vi "Replace Default with Tag.vi"(5 "instance id":string, 7 "engine configuration in":refnum<class "engine configuration.lvclass">, 9 "Channel Index":i32, 10 "Channel":refnum<class "TBM channel.lvclass">, 11 "Array in":string[](array[string])) -> (3 "Array out":string[](array[string]))   [LabVIEW 2015, in "PID Module configuration.lvclass"]
uses:
  module/configuration/PID Module configuration.lvclass
  <vilib>/NI/Module Execution Interface/Engine Configuration/engine configuration.lvclass
  <vilib>/NI/Tag Bus Module Framework/channel/TBM channel.lvclass
  <vilib>/NI/Module Execution Interface/Engine Configuration/unique channel identifier.ctl
  <vilib>/NI/Tag Bus/tag/tag descriptor.lvclass/tag descriptor.ctl
  <vilib>/NI/Module Execution Interface/Engine Configuration/engine configuration.lvclass/engine configuration.ctl
  <vilib>/NI/Tag Bus/tag/tag descriptor.lvclass
panel:
  out "readers":T1[](array[typedef])
  out "writer":T1
  out "Array":string[](array[string])
  out "name":string
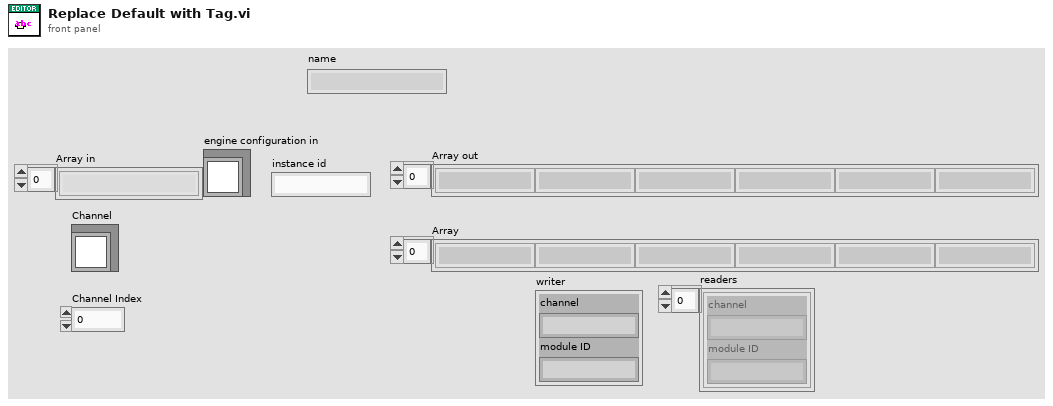
[diagram p1: front panel]
types:
  T1 = typedef "engine configuration.lvclass/unique channel identifier.ctl" = cluster{"channel":string, "module ID":string}
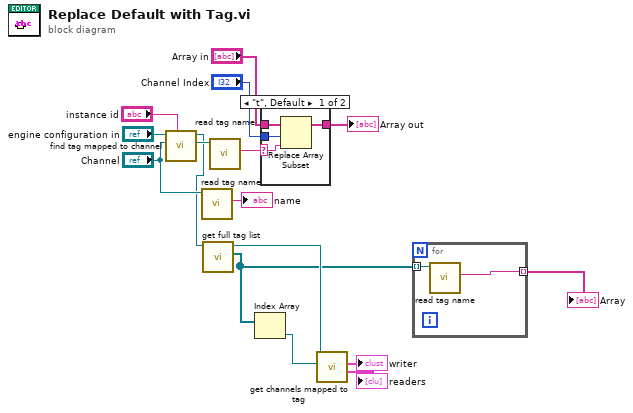
[diagram p0: block diagram]
diagram:
  n1 = call <vilib>:"find tag mapped to channel.vi"("owner"="instance id", "channel"="Channel", "engine configuration in"="engine configuration in") -> ("tag"=w15:refnum<class "tag descriptor.lvclass">, "engine configuration out"=w7:refnum<class "engine configuration.lvclass">)  [unwired: 6 in, 1 out]
  n2 = call <vilib>:"read tag name.vi"("system tag in"="Channel") -> ("name"=→"name":string)  [unwired: 8 in, 2 out]
  n3 = call <vilib>:"get full tag list.vi"("engine configuration in"=w7) -> ("tag list"=w4:refnum<class "tag descriptor.lvclass">[], "engine configuration out"=w5:refnum<class "engine configuration.lvclass">)  [unwired: 9 in]
  n4 = call <vilib>:"read tag name.vi"("system tag in"=w15) -> ("name"=w13:string)  [unwired: 8 in, 2 out]
  n5 = Index Array(array=w4) -> (element=w3:refnum<class "tag descriptor.lvclass">)  [unwired: 1 in]
  n6 = case shown="\"t\", Default" w13 {
    selector: w13 -> [w20 _]
    tunnel: [w18 w21] -> w12
    tunnel: "Array in" -> [w19 w21]
    tunnel: "Channel Index" -> [w17 _]
    frame "t", Default {
      n7 = Replace Array Subset(array=w19, new element=w20, index=w17) -> (w18:string[])
    }
    frame "" {
    }
  }
  "Array out" <- w12
  n8 = call-dynamic "get channels mapped to tag.vi"("tag"=w3, "engine configuration in"=w5) -> ("readers"=→"readers":T1[], "writer"=→"writer":T1)  [unwired: 6 in, 2 out]
  n9 = for {
    tunnel: w4 -> [w23] mode=indexing
    tunnel: [w22] -> w6 mode=indexing
    n10 = call <vilib>:"read tag name.vi"("system tag in"=w23) -> ("name"=w22:string)  [unwired: 8 in, 2 out]
  }
  "Array" <- w6
